vi "KYFG Set Camera Value Enum By Value Name.vi"(8 "error in (no error)":errorcluster, 9 "paramValueName":string, 10 "paramName":string, 11 "camHandle":u32) -> (0 "error out":errorcluster, 3 "camHandle out":u32)   [LabVIEW 2023, in "KYFGLib_lv.lvlib"]
doc: "KYFG_API FGSTATUS KYFG_SetCameraValueEnum_ByValueName(CAMHANDLE camHandle, const char *paramName, const char *paramValueName);"
uses:
  KYFGLib_lv.lvlib
  KYFGLib.dll
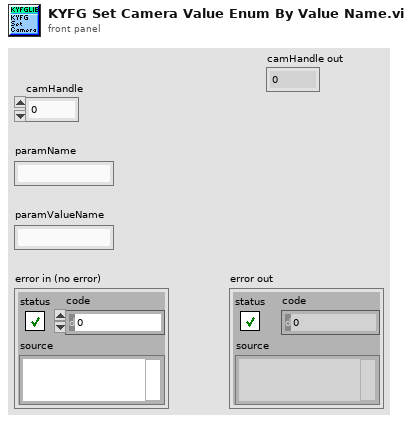
[diagram p1: front panel]
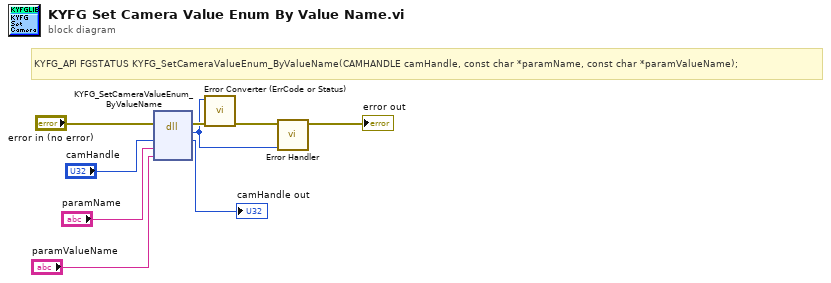
[diagram p0: block diagram]
diagram:
  # "KYFG_API FGSTATUS\tKYFG_SetCameraValueEnum_ByValueName(CAMHANDLE camHandle, const char *paramName, const char *paramValueName);"
  n1 = dll-call lib="KYFGLib.dll" fn="KYFG_SetCameraValueEnum_ByValueName"(error in="error in (no error)", "camHandle"="camHandle", "paramName"="paramName", "paramValueName"="paramValueName") -> (error out=w5:errorcluster, "return type"=w2:u32, "camHandle"=→"camHandle out":u32)  [unwired: 4 in, 1 out]
  n2 = call "Error Converter (ErrCode or Status).vi"("error in (no error)"=w5, "error code"=w2) -> ("error out"=w4:errorcluster)  [unwired: 9 in]
  n3 = call "Error Handler.vi"("Return Code"=w2, "Error In"=w4) -> ("Error Out"=→"error out":errorcluster)  [unwired: 9 in]
